vi "CarWashTestcase.vi"(11 "error in":errorcluster) -> (15 "error out":errorcluster)   [LabVIEW 2016, in "CarWashTest.lvlib"]
doc: "Perform test for Car Wash"
uses:
  CarWashTest.lvlib
  Controls/WashStepConfig.ctl
  <vilib>/addons/_JKI Toolkits/Caraya/classes/Test/Test.lvclass
panel:
  out "Wash Array":T1[](array[typedef])
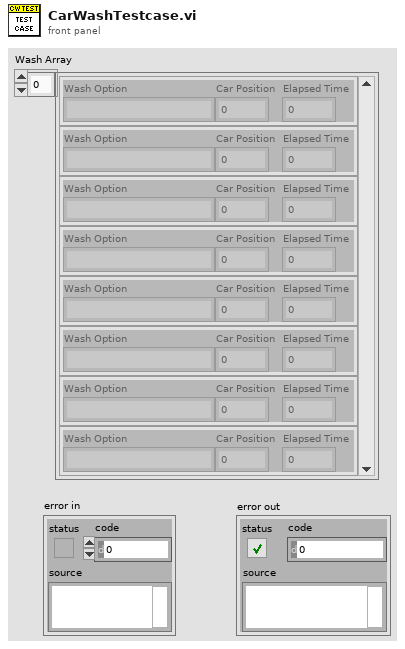
[diagram p1: front panel]
types:
  T1 = typedef "CarWashTest.lvlib/WashStepConfig.ctl" = cluster{"Wash Option":string, "Car Position":i32, "Elapsed Time":dbl}
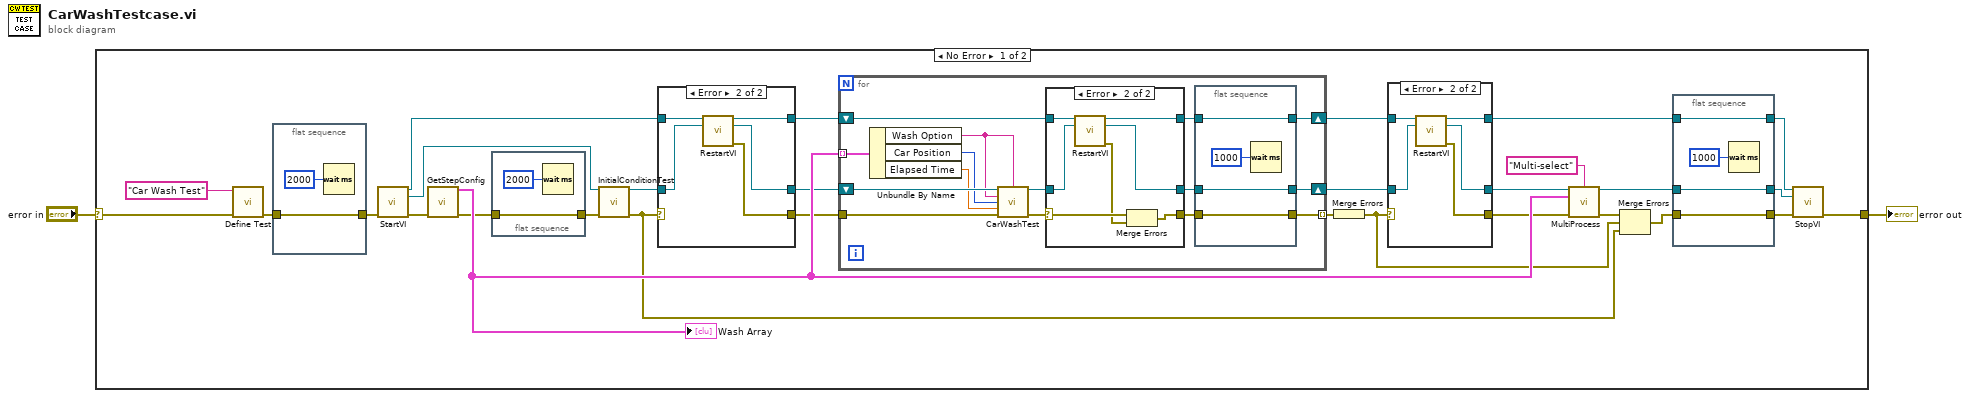
[diagram p0: block diagram]
diagram:
  n1 = case shown="No Error" "error in" {
    selector: "error in" -> [w6 w86]
    tunnel: [w3 w86] -> w1
    frame No Error {
      n2 = call <vilib>:"Define Test.vi"("error in (no error)"=w6, "Label (VI Title)"="Car Wash Test" ("Label")) -> ("error out"=w14:errorcluster)  [unwired: 8 in, 1 out]
      n3 = flat-sequence {
        tunnel: [w35] -> w29
        tunnel: w14 -> [w35]
        frame #0 {
          n4 = Wait (ms)(milliseconds to wait=u32 2000) -> ()  [unwired: 1 out]
        }
      }
      n5 = call "StartVI.vi"("error in"=w29) -> ("Application Ref out"=w30:refnum<vi>, "VI Reference"=w31:refnum<vi>, "error out"=w32:errorcluster)  [unwired: 12 in]
      n6 = call "GetStepConfig.vi"("error in"=w32) -> ("Wash Array"=w28:T1[], "error out"=w5:errorcluster)  [unwired: 13 in]
      "Wash Array" <- w28
      n7 = flat-sequence {
        tunnel: [w33] -> w4
        tunnel: w5 -> [w33]
        frame #0 {
          n8 = Wait (ms)(milliseconds to wait=u32 2000) -> ()  [unwired: 1 out]
        }
      }
      n9 = call "InitialConditionTest.vi"("VI Reference In"=w31, "error in"=w4) -> ("VI Reference Out"=w21:refnum<vi>, "error out"=w24:errorcluster)  [unwired: 12 in]
      n10 = case shown="Error" w24 {
        selector: w24 -> [w42 _]
        tunnel: [w42 w48] -> w27
        tunnel: w21 -> [w43 w46]
        tunnel: [w43 w47] -> w22
        tunnel: [w41 w44] -> w20
        tunnel: w30 -> [w41 w45]
        frame No Error {
        }
        frame Error {
          n11 = call "RestartVI.vi"("Application Ref in"=w45, "VI in"=w46) -> ("Application Ref out"=w44:refnum<vi>, "VI out"=w47:refnum<vi>, "error out"=w48:errorcluster)  [unwired: 11 in]
        }
      }
      n12 = for {
        shift-right: [w52] -> w16
        shift-left: w22 -> [w62]
        tunnel: w28 -> [w61] mode=indexing
        tunnel: w27 -> [w63]
        tunnel: [w55] -> w9 mode=indexing
        shift-right: [w51] -> w15
        shift-left: w20 -> [w49]
        n13 = Unbundle By Name(w61) -> ("Wash Option"=w58:string, "Car Position"=w60:i32, "Elapsed Time"=w59:dbl)
        n14 = call "CarWashTest.vi"("VI Reference In"=w62, "Label"=w58, "Wash Option"=w58, "Car Position"=w60, "Elapsed Time"=w59, "error in"=w63) -> ("VI Reference Out"=w56:refnum<vi>, "error out"=w57:errorcluster)  [unwired: 8 in]
        n15 = case shown="Error" w57 {
          selector: w57 -> [w69 w77]
          tunnel: [w69 w76] -> w54
          tunnel: w56 -> [w70 w74]
          tunnel: [w70 w71] -> w53
          tunnel: [w68 w72] -> w50
          tunnel: w49 -> [w68 w73]
          frame No Error {
          }
          frame Error {
            n16 = call "RestartVI.vi"("Application Ref in"=w73, "VI in"=w74) -> ("Application Ref out"=w72:refnum<vi>, "VI out"=w71:refnum<vi>, "error out"=w75:errorcluster)  [unwired: 11 in]
            n17 = Merge Errors(w77, w75) -> (w76:errorcluster)
          }
        }
        n18 = flat-sequence {
          tunnel: [w67] -> w55
          tunnel: w54 -> [w67]
          tunnel: w53 -> [w66]
          tunnel: [w66] -> w52
          tunnel: [w65] -> w51
          tunnel: w50 -> [w65]
          frame #0 {
            n19 = Wait (ms)(milliseconds to wait=u32 1000) -> ()  [unwired: 1 out]
          }
        }
      }
      n20 = Merge Errors(w9) -> (w25:errorcluster)
      n21 = case shown="Error" w25 {
        selector: w25 -> [w79 _]
        tunnel: [w79 w85] -> w19
        tunnel: w16 -> [w80 w83]
        tunnel: [w80 w84] -> w17
        tunnel: [w78 w81] -> w18
        tunnel: w15 -> [w78 w82]
        frame No Error {
        }
        frame Error {
          n22 = call "RestartVI.vi"("Application Ref in"=w82, "VI in"=w83) -> ("Application Ref out"=w81:refnum<vi>, "VI out"=w84:refnum<vi>, "error out"=w85:errorcluster)  [unwired: 11 in]
        }
      }
      n23 = call "MultiProcess.vi"("VI Reference In"=w17, "Label"="Multi-select", "Wash Array"=w28, "error in"=w19) -> ("VI Reference Out"=w10:refnum<vi>, "error out"=w26:errorcluster)  [unwired: 10 in]
      n24 = Merge Errors(w26, w25, w24) -> (w23:errorcluster)
      n25 = flat-sequence {
        tunnel: [w40] -> w13
        tunnel: w23 -> [w40]
        tunnel: w10 -> [w37]
        tunnel: [w39] -> w12
        tunnel: w18 -> [w39]
        tunnel: [w37] -> w11
        frame #0 {
          n26 = Wait (ms)(milliseconds to wait=u32 1000) -> ()  [unwired: 1 out]
        }
      }
      n27 = call "StopVI.vi"("Application Ref in"=w12, "VI in"=w11, "error in (no error)"=w13) -> ("error out"=w3:errorcluster)  [unwired: 12 in]
    }
    frame Error {
    }
  }
  "error out" <- w1
